vi "RDC-Lin-Calc_Permittivity.vi"(5 "C0":dbl format="%#_6p", 11 "input cluster":T1) -> (3 "Output cluster":T1)   [LabVIEW 2020, in "RDC-Reflection_Data_Computation.lvlib"]
doc: "Computes the permittivity of a Common Format cluster from its data and the probe capacitance C0, and returns the cluster with Permativity' and Permativity'' filled in."
uses:
  RDC-Reflection_Data_Computation.lvlib
  Reflector/RFH-common_data_format.ctl
  Reflector/RFH-Reflection_File_Handler.lvlib
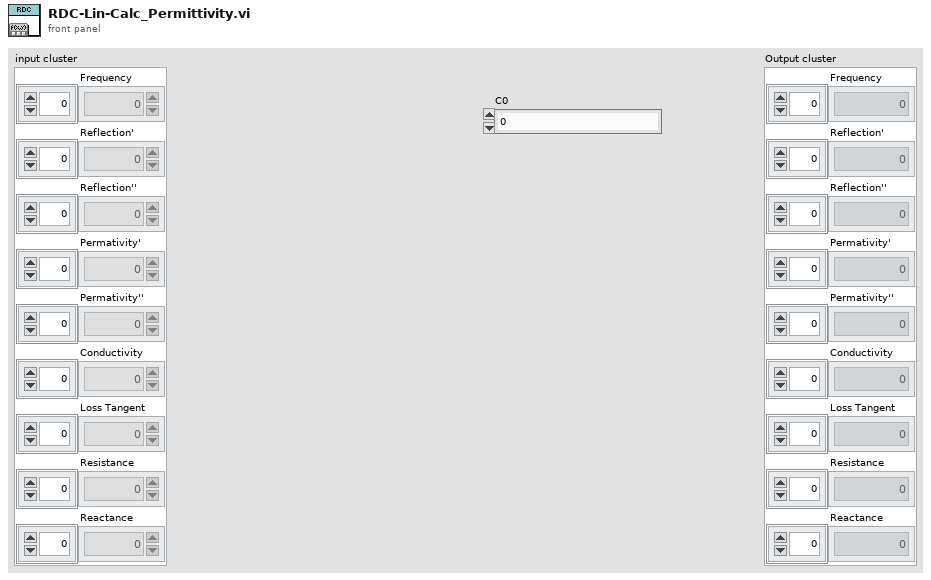
[diagram p1: front panel]
types:
  T1 = typedef "RFH-Reflection_File_Handler.lvlib/RFH-common_data_format.ctl" = cluster{"Frequency":dbl[], "Reflection'":dbl[], "Reflection''":dbl[], "Permativity'":dbl[], "Permativity''":dbl[], "Conductivity":dbl[], "Loss Tangent":dbl[], "Resistance":dbl[], "Reactance":dbl[]}
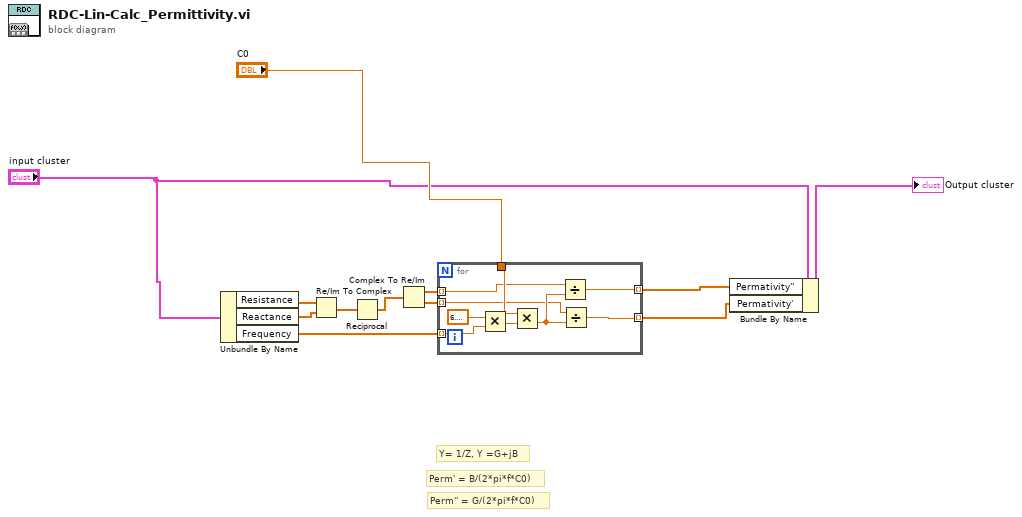
[diagram p0: block diagram]
diagram:
  # "Perm'' = G/(2*pi*f*C0)"
  # "Y= 1/Z, Y =G+jB"
  # "Perm' = B/(2*pi*f*C0)"
  n1 = Unbundle By Name("input cluster") -> ("Resistance"=w5:dbl[], "Reactance"=w4:dbl[], "Frequency"=w10:dbl[])
  n2 = Re/Im To Complex(1:w4, 2:w5) -> (0:w3:cdb[])
  n3 = Reciprocal(x=w3) -> (1/x=w2:cdb[])
  n4 = Complex To Re/Im(x + iy=w2) -> (x=w12:dbl[], y=w11:dbl[])
  n5 = for {
    tunnel: "C0" -> [w18]
    tunnel: w12 -> [w16] mode=indexing
    tunnel: w11 -> [w15] mode=indexing
    tunnel: w10 -> [w20] mode=indexing
    tunnel: [w14] -> w7 mode=indexing
    tunnel: [w13] -> w6 mode=indexing
    n6 = Multiply(x=6.283185307179586, y=w20) -> (x*y=w19:dbl)
    n7 = Multiply(x=w18, y=w19) -> (x*y=w17:dbl)
    n8 = Divide(x=w16, y=w17) -> (x/y=w14:dbl)
    n9 = Divide(x=w15, y=w17) -> (x/y=w13:dbl)
  }
  n10 = Bundle By Name(cluster="input cluster", "Permativity''"=w7, "Permativity'"=w6) -> (→"Output cluster":T1)
